vi "Module Loop.vi"(8 "error in (no error)":errorcluster, 11 "ValveSimModule in":refnum<class "ValveSimModule.lvclass">) -> (0 "error out":errorcluster, 3 "ValveSimModule out":refnum<class "ValveSimModule.lvclass">)   [LabVIEW 2020, in "VolatusScratch.lvlib" / "ValveSimModule.lvclass"]
uses:
  ValveSimModule.lvclass
  C:/dev/lv20CE/relink/lv-volatus/Volatus/Module/Module.lvclass
  Valve State.ctl
  Volatus/Module/Module.lvclass
  ValveSimModule.lvclass/ValveSimModule.ctl
  Volatus/Module/Module.lvclass/Module.ctl
  Volatus/VolatusAPI/VolatusAPI.lvclass/VolatusAPI.ctl
  messages/CmdDigital/Class/Msg.lvclass
  C:/dev/lv20CE/relink/lv-protoc/LV-Proto/Message/Message.lvclass
  messages/CmdDigital/Class/Msg.lvclass/Msg.ctl
  lv-vecto/Vecto/Channel DBL/Channel DBL.lvclass/Channel DBL.ctl
  lv-vecto/Vecto/Group DBL/Group DBL.lvclass
  C:/dev/lv20CE/relink/lv-vecto/Vecto/Group/Group.lvclass
  lv-vecto/Vecto/Group DBL/Update Value by Index.vi
  <vilib>/Utility/error.llb/Error Cluster From Error Code.vi
  lv-vecto/Vecto/Vecto.lvlib
  lv-vecto/Vecto/Channel DBL/Channel DBL.lvclass
panel:
  in  "Both Limits":bool
  out "State":T1
  in  "Skip Publish":bool
  out "Energized":bool
  out "Open":bool
  out "Closed":bool
  out "Command":bool
  in  "Energize Delay":dbl=0.3
  in  "Close Time":dbl=0.8
  in  "Open Time":dbl=0.6
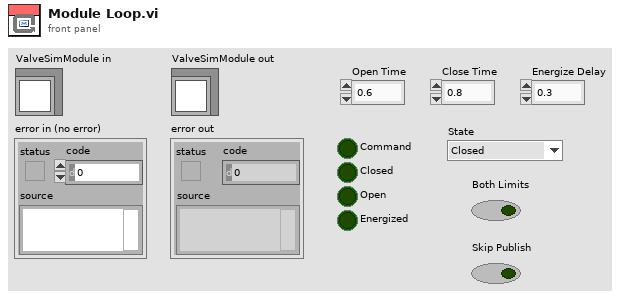
[diagram p1: front panel]
types:
  T1 = typedef "VolatusScratch.lvlib/ValveSimModule.lvclass/Valve State.ctl" = enum16{"Closed", "Energize", "Open", "Opened", "Deenergize", "Close"}
  T2 = cluster{"Open Time":dbl, "Close Time":dbl, "Energize Delay":dbl}
  T3 = typedef "CmdDigital.lvlib/Data.ctl" = cluster{"channel":string, "value":bool}
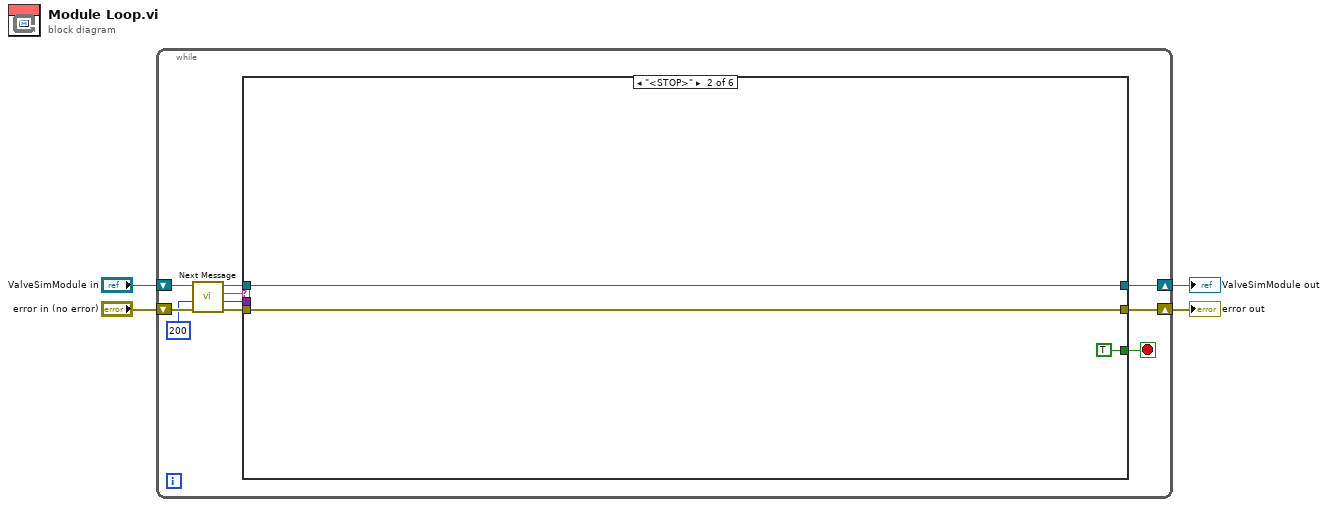
[diagram p0: block diagram]
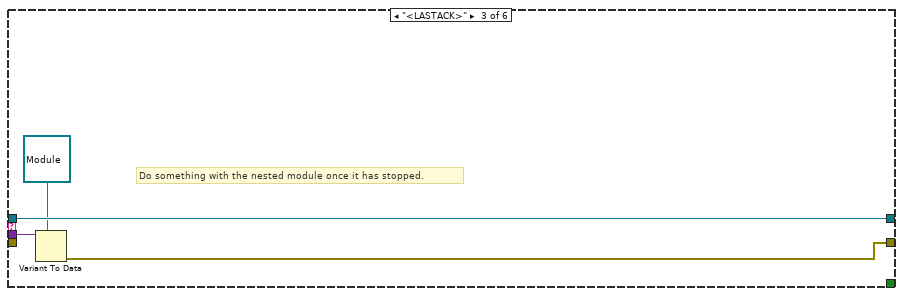
[diagram p3: hidden frame]
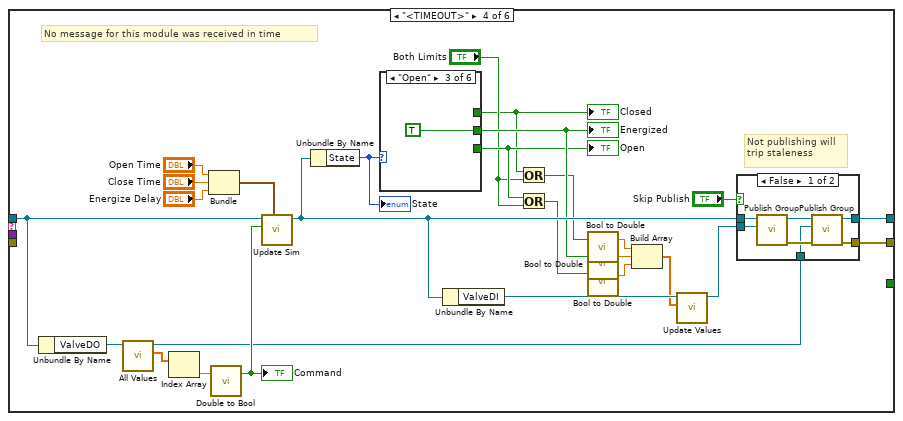
[diagram p4: hidden frame]
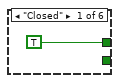
[diagram p6: hidden frame]
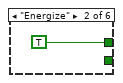
[diagram p7: hidden frame]
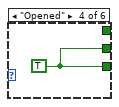
[diagram p8: hidden frame]
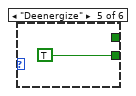
[diagram p9: hidden frame]
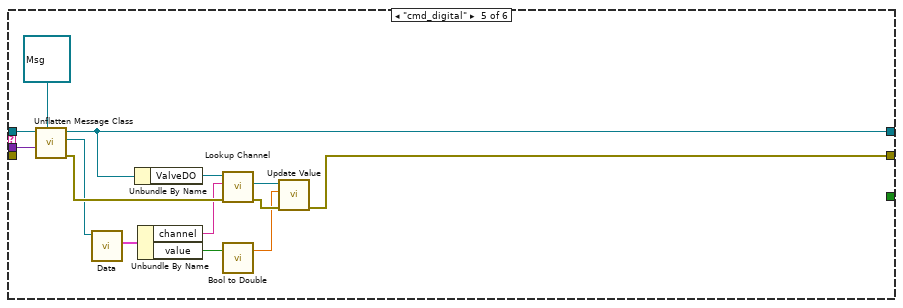
[diagram p11: hidden frame]
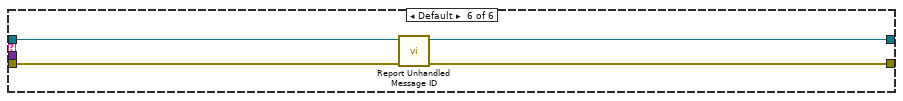
[diagram p12: hidden frame]
diagram:
  n1 = while {
    shift-right: [w9] -> w2
    shift-left: "ValveSimModule in" -> [w14]
    shift-right: [w8] -> w1
    shift-left: "error in (no error)" -> [w13]
    stop <- w7 stop-if-true
    n2 = call "Next Message.vi"("error in (no error)"=w13, "Timeout ms (-1)"=200, "Module in"=w14) -> ("error out"=w12:errorcluster, "Data"=w6:variant, "ID"=w11:string, "Module out"=w10:refnum<class "ValveSimModule.lvclass">)  [unwired: 5 in]
    n3 = case shown="\"<STOP>\"" w11 {
      tunnel: w12 -> [w15 w18 _ _ _ w81]
      tunnel: w10 -> [w16 w19 w23 w50 w76 w79]
      tunnel: [w16 w19 w23 w33 w71 w78] -> w9
      tunnel: [w15 w18 w20 w31 w64 w80] -> w8
      tunnel: [_ TRUE _ _ _ _] -> w7
      tunnel: w6 -> [_ _ w22 _ w74 _]
      frame "<CLOSE>" {
      }
      frame "<STOP>" {
      }
      frame "<LASTACK>" {
        # "Do something with the nested module once it has stopped."
        n4 = Variant To Data(type=refnum<class "Module.lvclass"> refnum ("Volatus:Module"), Variant=w22) -> (error out=w20:errorcluster)  [unwired: 1 in, 1 out]
      }
      frame "<TIMEOUT>" {
        # "Not publishing will trip staleness"
        # "No message for this module was received in time"
        n5 = Unbundle By Name(w50) -> ("ValveDO"=w49:refnum<class "Group DBL.lvclass">)
        n6 = call "All Values.vi"("Group in"=w49) -> ("Scaled"=w48:dbl[], "Group out"=w32:refnum<class "Group DBL.lvclass">)  [unwired: 6 in, 3 out]
        n7 = Index Array(array=w48) -> (element=w47:dbl)  [unwired: 1 in]
        n8 = Bundle("Open Time"="Open Time", "Close Time"="Close Time", "Energize Delay"="Energize Delay") -> (w42:T2)  [unwired: 1 in]
        n9 = call "Double to Bool.vi"("Double"=w47) -> ("Bool"=w46:bool)  [unwired: 2 in]
        "Command" <- w46
        n10 = call "Update Sim.vi"("Timings"=w42, "Command"=w46, "ValveSimModule in"=w50) -> ("ValveSimModule out"=w40:refnum<class "ValveSimModule.lvclass">)  [unwired: 7 in, 1 out]
        n11 = Unbundle By Name(w40) -> ("State"=w41:T1)
        "State" <- w41
        n12 = case shown="\"Open\"" w41 {
          tunnel: [TRUE TRUE _ _ _ _] -> w25
          tunnel: [_ _ TRUE w62 _ _] -> w29
          tunnel: [_ _ _ w62 TRUE _] -> w28
          frame "Closed" {
          }
          frame "Energize" {
          }
          frame "Open" {
          }
          frame "Opened" {
            w62 = TRUE
          }
          frame "Deenergize" {
          }
          frame "Close" {
          }
        }
        "Closed" <- w25
        "Open" <- w28
        "Energized" <- w29
        n13 = Unbundle By Name(w40) -> ("ValveDI"=w36:refnum<class "Group DBL.lvclass">)
        n14 = Or(x=w25, y="Both Limits") -> (x .or. y?=w24:bool)
        n15 = Or(x=w28, y="Both Limits") -> (x .or. y?=w27:bool)
        n16 = call "Bool to Double.vi"("Bool"=w24) -> ("Double"=w39:dbl)  [unwired: 2 in]
        n17 = call "Bool to Double.vi"("Bool"=w29) -> ("Double"=w38:dbl)  [unwired: 2 in]
        n18 = call "Bool to Double.vi"("Bool"=w27) -> ("Double"=w37:dbl)  [unwired: 2 in]
        n19 = Build Array(w39, w38, w37) -> (w35:dbl[])
        n20 = call "Update Values.vi"("Values"=w35, "Group in"=w36) -> ("Group out"=w34:refnum<class "Group DBL.lvclass">)  [unwired: 8 in, 1 out]
        n21 = case shown="False" "Skip Publish" {
          tunnel: w40 -> [w56 w58]
          tunnel: w34 -> [w54 _]
          tunnel: [w53 w58] -> w33
          tunnel: w32 -> [w52 _]
          tunnel: [w51 _] -> w31
          frame False {
            n22 = call "Publish Group.vi"("Group"=w54, "Module in"=w56) -> ("error out"=w57:errorcluster, "Module out"=w55:refnum<class "ValveSimModule.lvclass">)  [unwired: 8 in]
            n23 = call "Publish Group.vi"("error in (no error)"=w57, "Group"=w52, "Module in"=w55) -> ("error out"=w51:errorcluster, "Module out"=w53:refnum<class "ValveSimModule.lvclass">)  [unwired: 7 in]
          }
          frame True {
          }
        }
      }
      frame "cmd_digital" {
        n24 = call "Unflatten Message Class.vi"("Message Type"=refnum<class "Msg.lvclass"> refnum ("CmdDigital.lvlib:Msg.lvclass"), "Data"=w74, "Module in"=w76) -> ("error out"=w77:errorcluster, "Message"=w73:refnum<class "Msg.lvclass">, "Module out"=w71:refnum<class "ValveSimModule.lvclass">)  [unwired: 5 in, 1 out]
        n25 = call "Data.vi"("PB Msg Template in"=w73) -> ("Data"=w72:T3)  [unwired: 8 in, 2 out]
        n26 = Unbundle By Name(w71) -> ("ValveDO"=w70:refnum<class "Group DBL.lvclass">)
        n27 = Unbundle By Name(w72) -> ("channel"=w69:string, "value"=w67:bool)
        n28 = call "Lookup Channel.vi"("error in (no error)"=w77, "Channel Name"=w69, "Group in"=w70) -> ("error out"=w66:errorcluster, "Channel"=w68:refnum<class "Channel DBL.lvclass">)  [unwired: 6 in, 1 out]
        n29 = call "Bool to Double.vi"("Bool"=w67) -> ("Double"=w65:dbl)  [unwired: 2 in]
        n30 = call "Update Value.vi"("error in (no error)"=w66, "Value"=w65, "Channel in"=w68) -> ("error out"=w64:errorcluster)  [unwired: 7 in, 1 out]
      }
      frame Default {
        n31 = call "Report Unhandled Message ID.vi"("error in (no error)"=w81, "Module in"=w79) -> ("error out"=w80:errorcluster, "Module out"=w78:refnum<class "ValveSimModule.lvclass">)  [unwired: 8 in]
      }
    }
  }
  "error out" <- w1
  "ValveSimModule out" <- w2
